vi "display Axis Parameter List.vi"(8 "error in (no error)":errorcluster, 11 "VISA resource name":refnum<visa-resource-name>) -> (0 "error out":errorcluster, 1 "Position Info":T1, 3 "VISA resource name out":refnum<visa-resource-name>)   [LabVIEW 2023, in "FCC 3D Controller for BS.lvlib"]
uses:
  <vilib>/Utility/error.llb/Trim Whitespace One-Sided.vi
  FCC 3D Controller for BS.lvlib
panel:
  out "read buffer 8":string
  out "Limit Negative String":string
  out "Limit Positive String":string
  out "Current Position":string
  out "Target Position":string
  out "Velocity String":string
  out "read buffer":string
  out "read buffer 7":string
  out "read buffer 6":string
  out "read buffer 5":string
  out "read buffer 4":string
  out "read buffer 3":string
  out "read buffer 2":string
  out "Acc/Deceleration String":string
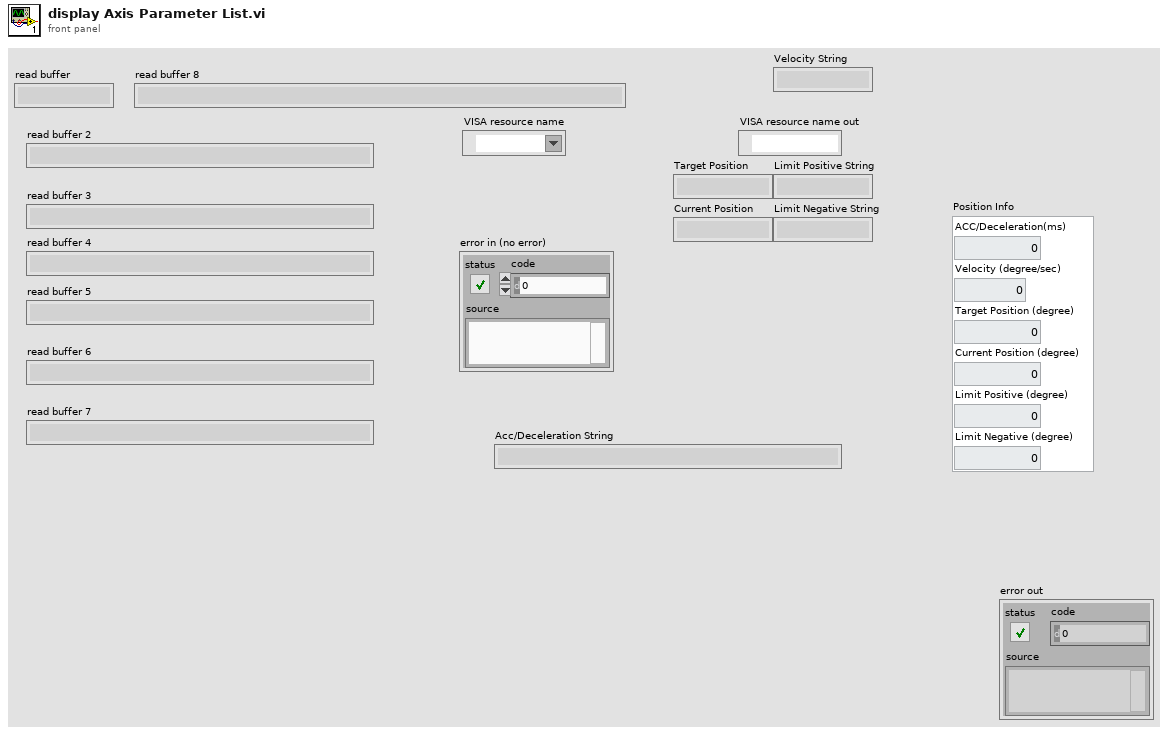
[diagram p1: front panel]
types:
  T1 = cluster{"ACC/Deceleration(ms)":dbl, "Velocity (degree/sec)":dbl, "Target Position (degree)":dbl, "Current Position (degree)":dbl, "Limit Positive (degree)":dbl, "Limit Negative (degree)":dbl}
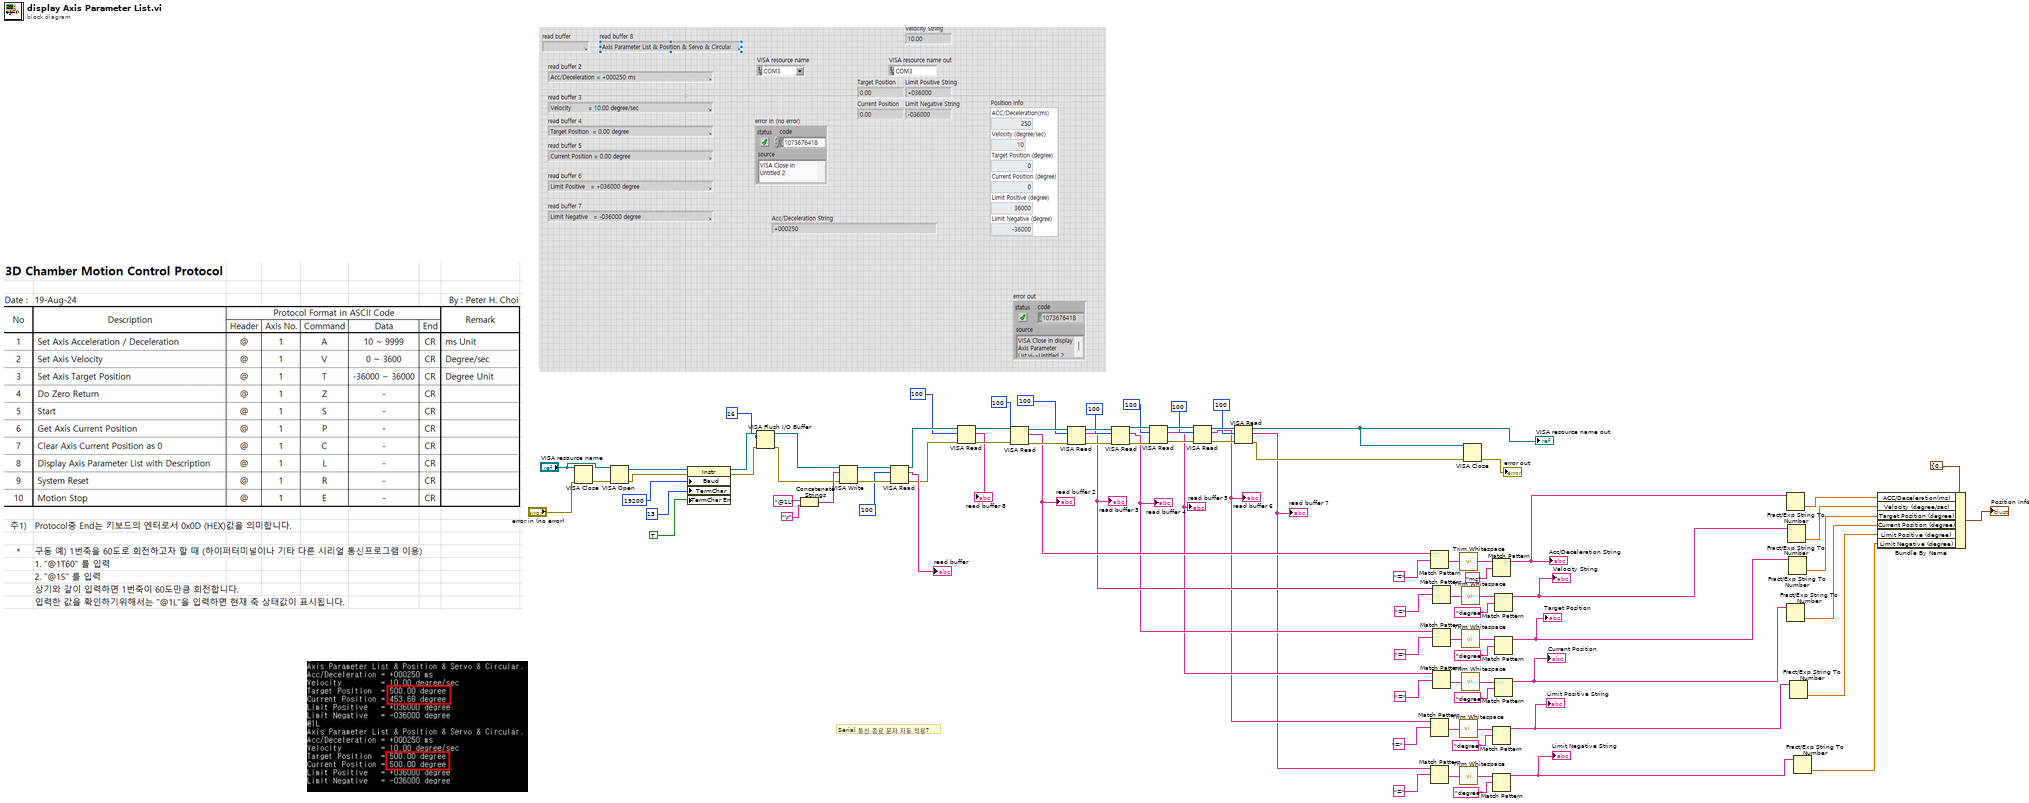
[diagram p0: block diagram]
diagram:
  # "Serial 통신 종료 문자 자동 적용?"
  n1 = VISA Close(VISA resource name="VISA resource name", error in (no error)="error in (no error)") -> (error out=w84:errorcluster)
  n2 = VISA Open(error in (no error)=w84, VISA resource name="VISA resource name") -> (VISA resource name=w80:refnum<visa-resource-name>, error out=w78:errorcluster)  [unwired: 3 in]
  n3 = property class="Instr"(reference=w80, error in=w78, "Baud"=u32 19200 ("Serial Settings:Baud Rate"), "TermChar"=u8 13 ("Message Based Settings:Termination Character"), "TermChar En"=TRUE ("Message Based Settings:Termination Character Enable")) -> (reference out=w68:refnum<visa-resource-name>, error out=w66:errorcluster)
  n4 = VISA Flush I/O Buffer(VISA resource name=w68, mask (16)=u16 16, error in (no error)=w66) -> (VISA resource name out=w67:refnum<visa-resource-name>, error out=w65:errorcluster)
  n5 = Concatenate Strings("@1L" ("write buffer"), "\r") -> (w73:string)
  n6 = VISA Write(VISA resource name=w67, write buffer=w73, error in (no error)=w65) -> (VISA resource name out=w82:refnum<visa-resource-name>, error out=w81:errorcluster)  [unwired: 1 out]
  n7 = VISA Read(VISA resource name=w82, byte count=u32 100, error in (no error)=w81) -> (VISA resource name out=w6:refnum<visa-resource-name>, read buffer=→"read buffer":string, error out=w4:errorcluster)  [unwired: 1 out]
  n8 = VISA Read(VISA resource name=w6, byte count=u32 100, error in (no error)=w4) -> (VISA resource name out=w5:refnum<visa-resource-name>, read buffer=→"read buffer 8":string, error out=w3:errorcluster)  [unwired: 1 out]
  n9 = VISA Read(VISA resource name=w5, byte count=u32 100, error in (no error)=w3) -> (VISA resource name out=w70:refnum<visa-resource-name>, read buffer=w46:string, error out=w55:errorcluster)  [unwired: 1 out]
  "read buffer 2" <- w46
  n10 = VISA Read(VISA resource name=w70, byte count=u32 100, error in (no error)=w55) -> (VISA resource name out=w63:refnum<visa-resource-name>, read buffer=w39:string, error out=w54:errorcluster)  [unwired: 1 out]
  "read buffer 3" <- w39
  n11 = VISA Read(VISA resource name=w63, byte count=u32 100, error in (no error)=w54) -> (VISA resource name out=w61:refnum<visa-resource-name>, read buffer=w32:string, error out=w53:errorcluster)  [unwired: 1 out]
  "read buffer 4" <- w32
  n12 = VISA Read(VISA resource name=w61, byte count=u32 100, error in (no error)=w53) -> (VISA resource name out=w59:refnum<visa-resource-name>, read buffer=w26:string, error out=w52:errorcluster)  [unwired: 1 out]
  "read buffer 5" <- w26
  n13 = VISA Read(VISA resource name=w59, byte count=u32 100, error in (no error)=w52) -> (VISA resource name out=w57:refnum<visa-resource-name>, read buffer=w16:string, error out=w51:errorcluster)  [unwired: 1 out]
  "read buffer 6" <- w16
  n14 = VISA Read(VISA resource name=w57, byte count=u32 100, error in (no error)=w51) -> (VISA resource name out=w49:refnum<visa-resource-name>, read buffer=w9:string, error out=w48:errorcluster)  [unwired: 1 out]
  "VISA resource name out" <- w49
  "read buffer 7" <- w9
  n15 = Match Pattern(string=w16, regular expression="=") -> (after substring=w19:string)  [unwired: 1 in, 3 out]
  n16 = Match Pattern(string=w46, regular expression="=") -> (after substring=w87:string)  [unwired: 1 in, 3 out]
  n17 = Match Pattern(string=w9, regular expression="=") -> (after substring=w11:string)  [unwired: 1 in, 3 out]
  n18 = Match Pattern(string=w39, regular expression="=") -> (after substring=w41:string)  [unwired: 1 in, 3 out]
  n19 = Match Pattern(string=w32, regular expression="=") -> (after substring=w35:string)  [unwired: 1 in, 3 out]
  n20 = Match Pattern(string=w26, regular expression="=") -> (after substring=w28:string)  [unwired: 1 in, 3 out]
  n21 = call <vilib>:"Trim Whitespace.vi"("string"=w19) -> ("trimmed string"=w17:string)  [unwired: 1 in]
  n22 = call <vilib>:"Trim Whitespace.vi"("string"=w87) -> ("trimmed string"=w44:string)  [unwired: 1 in]
  n23 = call <vilib>:"Trim Whitespace.vi"("string"=w11) -> ("trimmed string"=w13:string)  [unwired: 1 in]
  n24 = call <vilib>:"Trim Whitespace.vi"("string"=w41) -> ("trimmed string"=w43:string)  [unwired: 1 in]
  n25 = call <vilib>:"Trim Whitespace.vi"("string"=w35) -> ("trimmed string"=w33:string)  [unwired: 1 in]
  n26 = call <vilib>:"Trim Whitespace.vi"("string"=w28) -> ("trimmed string"=w30:string)  [unwired: 1 in]
  n27 = VISA Close(VISA resource name=w49, error in (no error)=w48) -> (error out=→"error out":errorcluster)
  n28 = Match Pattern(string=w17, regular expression="degree") -> (before substring=w14:string)  [unwired: 1 in, 3 out]
  "Limit Positive String" <- w14
  n29 = Match Pattern(string=w44, regular expression="ms") -> (before substring=w85:string)  [unwired: 1 in, 3 out]
  "Acc/Deceleration String" <- w85
  n30 = Match Pattern(string=w13, regular expression="degree") -> (before substring=w7:string)  [unwired: 1 in, 3 out]
  "Limit Negative String" <- w7
  n31 = Match Pattern(string=w43, regular expression="degree") -> (before substring=w38:string)  [unwired: 1 in, 3 out]
  "Velocity String" <- w38
  n32 = Match Pattern(string=w33, regular expression="degree") -> (before substring=w31:string)  [unwired: 1 in, 3 out]
  "Target Position" <- w31
  n33 = Match Pattern(string=w30, regular expression="degree") -> (before substring=w21:string)  [unwired: 1 in, 3 out]
  "Current Position" <- w21
  n34 = Fract/Exp String To Number(string=w85) -> (number=w45:dbl)  [unwired: 3 in, 1 out]
  n35 = Fract/Exp String To Number(string=w21) -> (number=w24:dbl)  [unwired: 3 in, 1 out]
  n36 = Fract/Exp String To Number(string=w38) -> (number=w37:dbl)  [unwired: 3 in, 1 out]
  n37 = Fract/Exp String To Number(string=w31) -> (number=w25:dbl)  [unwired: 3 in, 1 out]
  n38 = Fract/Exp String To Number(string=w14) -> (number=w15:dbl)  [unwired: 3 in, 1 out]
  n39 = Fract/Exp String To Number(string=w7) -> (number=w8:dbl)  [unwired: 3 in, 1 out]
  n40 = Bundle By Name(cluster=T1 {"ACC/Deceleration(ms)"=0.0, "Velocity (degree/sec)"=0.0, "Target Position (degree)"=0.0, "Current Position (degree)"=0.0, "Limit Positive (degree)"=0.0, "Limit Negative (degree)"=0.0} ("Position Info"), "ACC/Deceleration(ms)"=w45, "Velocity (degree/sec)"=w37, "Target Position (degree)"=w25, "Current Position (degree)"=w24, "Limit Positive (degree)"=w15, "Limit Negative (degree)"=w8) -> (→"Position Info":T1)
